vi "query HO BandWidth.vi"(8 "error in (no error)":errorcluster caption="에러 입력(에러 없음)", 9 "LTE Channel Type":T2, 11 "LTE 입력":refnum<class "LTE.lvclass">) -> (0 "error out":errorcluster caption="에러 출력", 2 "BandWidth":T1, 3 "LTE 출력":refnum<class "LTE.lvclass">)   [LabVIEW 2023, in "ANRITSU Call Box.lvlib" / "LTE.lvclass"]
uses:
  LTE.lvclass
  LTE.lvclass/LTE.ctl
  ANRITSU Call Box.lvlib
  Type Definition/LTE Supported BandWidth.ctl
  Type Definition/LTE Channel Type.ctl
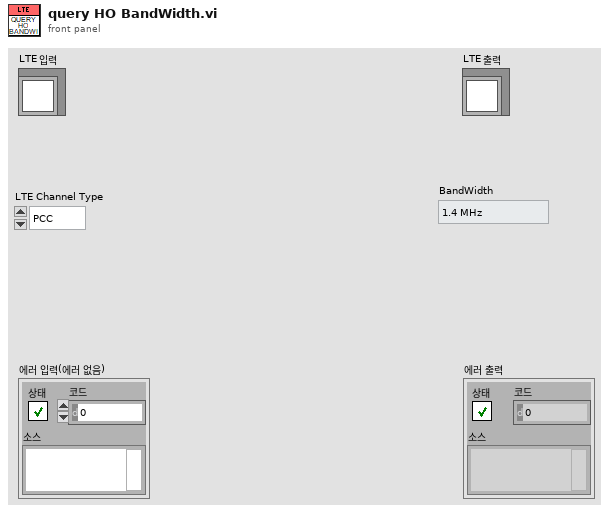
[diagram p1: front panel]
types:
  T1 = typedef "ANRITSU Call Box.lvlib/LTE Supported BandWidth.ctl" = enum16{"1.4 MHz", "3 MHz", "5 MHz", "10 MHz", "15 MHz", "20 MHz"}
  T2 = typedef "ANRITSU Call Box.lvlib/LTE Channel Type.ctl" = enum16{"PCC", "SCC1", "SCC2", "SCC3"}
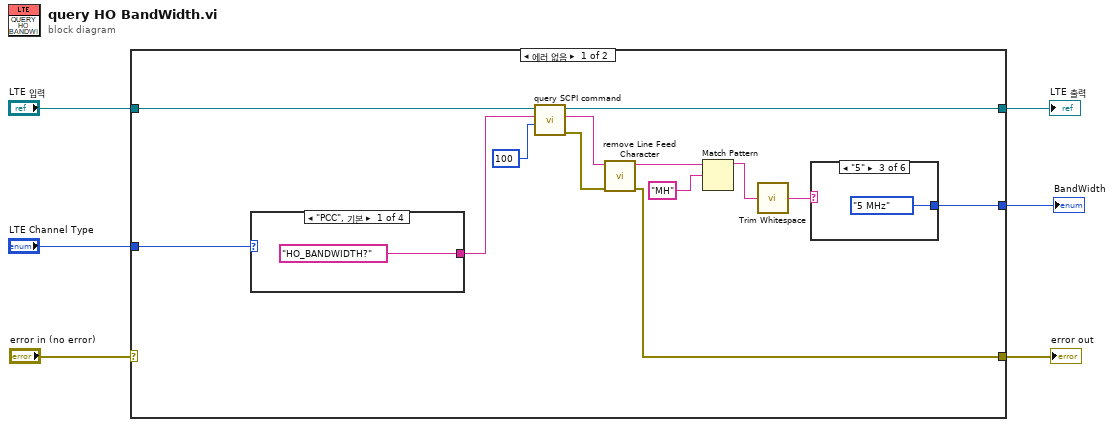
[diagram p0: block diagram]
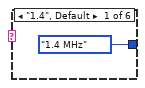
[diagram p2: hidden frame]
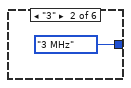
[diagram p3: hidden frame]
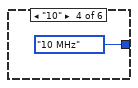
[diagram p4: hidden frame]
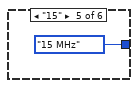
[diagram p5: hidden frame]
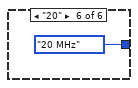
[diagram p6: hidden frame]
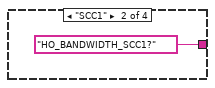
[diagram p7: hidden frame]
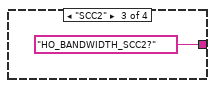
[diagram p8: hidden frame]
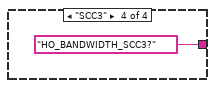
[diagram p9: hidden frame]
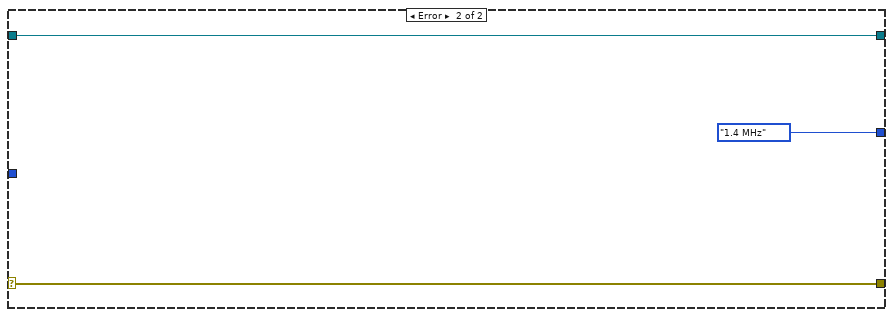
[diagram p10: hidden frame]
diagram:
  n1 = case shown="에러 없음" "error in (no error)" {
    selector: "error in (no error)" -> [_ w32]
    tunnel: [w7 w32] -> w5
    tunnel: [w9 w31] -> w3
    tunnel: "LTE 입력" -> [w10 w31]
    tunnel: "LTE Channel Type" -> [w11 _]
    tunnel: [w8 LTE_Supported_BandWidth."1.4 MHz" ("BandWidth 2")] -> w1
    frame No Error {
      n2 = case shown="\"PCC\", 기본" w11 {
        tunnel: ["HO_BANDWIDTH?" ("string") "HO_BANDWIDTH_SCC1?" ("string") "HO_BANDWIDTH_SCC2?" ("string") "HO_BANDWIDTH_SCC3?" ("string")] -> w19
        frame "PCC", Default {
        }
        frame "SCC1" {
        }
        frame "SCC2" {
        }
        frame "SCC3" {
        }
      }
      n3 = call "query SCPI command.vi"("Read Buffer Length"=u32 100, "SCPI Command"=w19, "LTE in"=w10) -> ("error out"=w16:errorcluster, "Read Buffer String"=w17:string, "LTE out"=w9:refnum<class "LTE.lvclass">)  [unwired: 6 in]
      n4 = call "remove Line Feed Character.vi"("error in"=w16, "Query String"=w17) -> ("error out"=w7:errorcluster, "Line Feed Removed String"=w15:string)  [unwired: 8 in]
      n5 = Match Pattern(string=w15, regular expression="MH") -> (before substring=w13:string)  [unwired: 1 in, 3 out]
      n6 = call <vilib>:"Trim Whitespace.vi"("string"=w13) -> ("trimmed string"=w12:string)  [unwired: 1 in]
      n7 = case shown="\"5\"" w12 {
        tunnel: [LTE_Supported_BandWidth."1.4 MHz" ("BandWidth 2") LTE_Supported_BandWidth."3 MHz" ("BandWidth 2") LTE_Supported_BandWidth."5 MHz" ("BandWidth 2") LTE_Supported_BandWidth."10 MHz" ("BandWidth 2") LTE_Supported_BandWidth."15 MHz" ("BandWidth 2") LTE_Supported_BandWidth."20 MHz" ("BandWidth 2")] -> w8
        frame "1.4", Default {
        }
        frame "3" {
        }
        frame "5" {
        }
        frame "10" {
        }
        frame "15" {
        }
        frame "20" {
        }
      }
    }
    frame Error {
    }
  }
  "error out" <- w5
  "LTE 출력" <- w3
  "BandWidth" <- w1
